vi "Global 1.vi"() -> ()   [LabVIEW 2024]
panel:
  in  "Initial":string[](array[string])
  in  "Rate of change":T1(array[cluster])
  out "Array 4":T2(array[cluster])
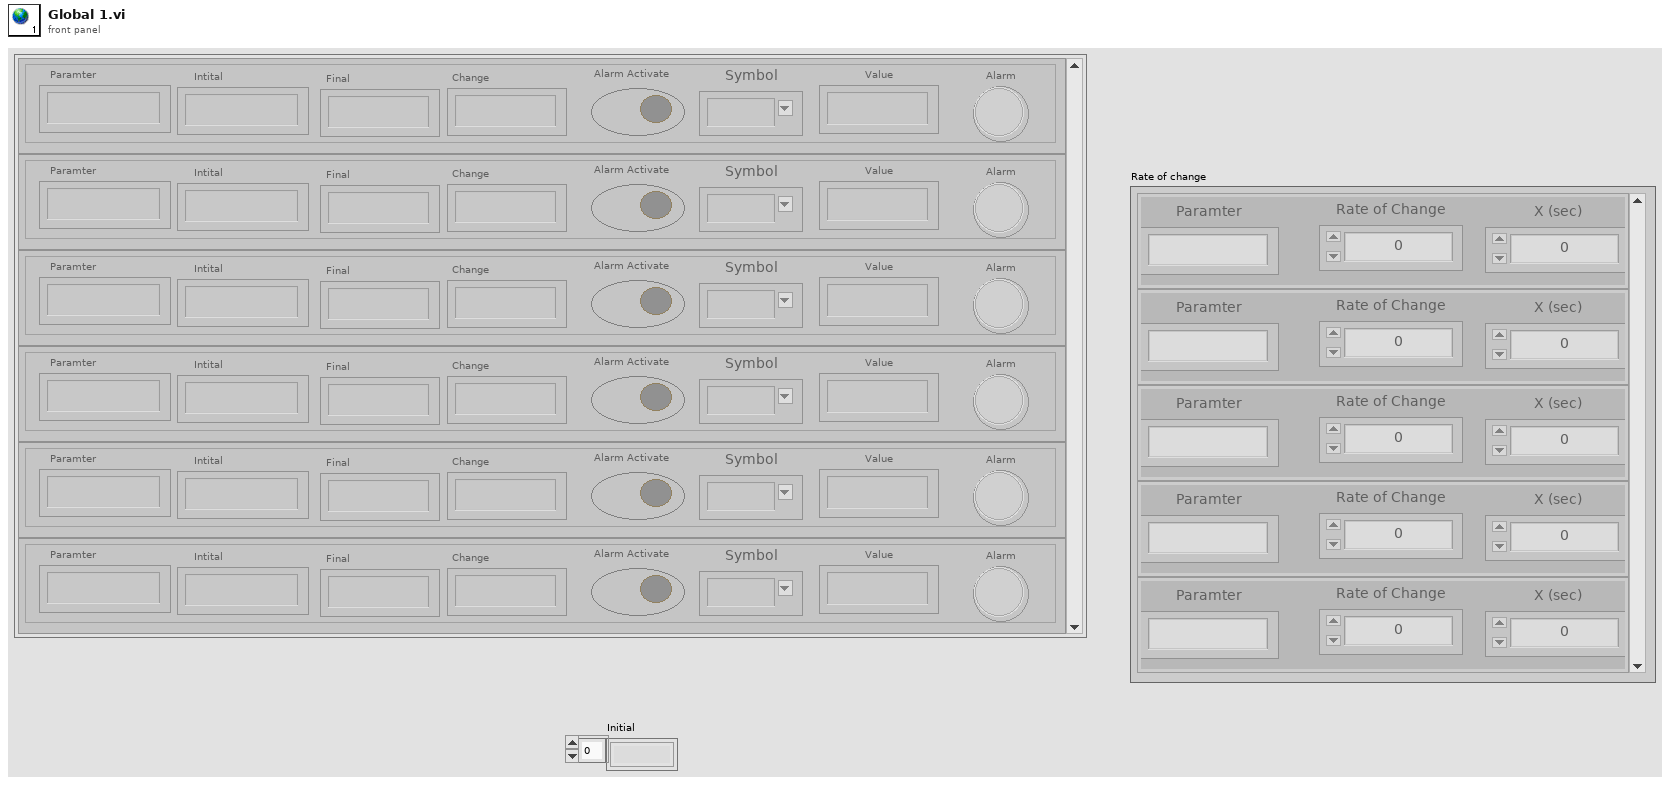
[diagram p1: front panel]
types:
  T1 = cluster{"Paramter":string, "Rate of Change":dbl, "X (sec)":dbl}[]
  T2 = cluster{"Paramter":string, "Intital ":string, "Final":string, "Change":string, "Alarm Activate ":bool, "Symbol":string, "Value":string, "Alarm":bool}[]
diagram:
